vi "SMR_LabVIEW_V10.vi"() -> ()   [LabVIEW 2025]
uses:
  <vilib>/DAQmx/write.llb/DAQmx Write (Analog DBL 1Chan 1Samp).vi
  <vilib>/DAQmx/read.llb/DAQmx Read (Analog 1D DBL NChan 1Samp).vi
  <vilib>/DAQmx/read.llb/DAQmx Read (Analog 2D DBL NChan NSamp).vi
  <vilib>/Analysis/baseanly.llb/Mean (DBL).vi
  <vilib>/DAQmx/create/channels.llb/DAQmx Create Channel (AI-Temperature-Thermocouple).vi
  <vilib>/DAQmx/create/channels.llb/DAQmx Create Channel (AI-Voltage-Basic).vi
  <vilib>/DAQmx/create/channels.llb/DAQmx Create Channel (AO-Voltage-Basic).vi
  <vilib>/DAQmx/miscellaneous.llb/DAQmx Fill In Error Info.vi
  <vilib>/DAQmx/configure/timing.llb/DAQmx Timing (Sample Clock).vi
  <vilib>/DAQmx/create/channels.llb/DAQmx Create Channel (AO-Current-Basic).vi
  <vilib>/addons/control/pid/pid.llb/PID (DBL).vi
  <vilib>/measure/maspectr.llb/FFT Power Spectrum and PSD for 1 Chan.vi
  <vilib>/measure/matone.llb/Extract Single Tone Information 1 Chan.vi
  <vilib>/addons/control/pid/pid.llb/PID Advanced (DBL).vi
  <vilib>/addons/control/pid/NI_PID_pid.lvlib
  <vilib>/Analysis/NI_AALBase.lvlib
  <vilib>/ptbypt/NI_PtbyPt.lvlib
  <vilib>/measure/NI_MAPro.lvlib
panel:
  out "HX Flow (GPM)":dbl
  out "HW Valve Command (V)":dbl
  in  "HX Flow Setpoint (GPM)":dbl
  in  "Manual HW Valve Command (V)":dbl min=0.0 max=10.0
  in  "HW Valve: Manual / PID (on)":bool
  out "Rod Power (W)":dbl
  in  "Resistance Burden (Ohm)":dbl=220.0 min=220.0 max=220.0
  out "PSU Command (mA)":dbl
  in  "PSU Power Setpoint (W)":dbl
  in  "Manual PSU Command (0-8.8)":dbl min=0.0 max=8.8
  in  "PSU: Manual/ PID (on)":bool
  in  "PID gains for PSU":T1={"proportional gain (Kc)"=0.0003, "integral time (Ti, min)"=0.025, "derivative time (Td, min)"=0.0} {"derivative time (Td, min)" format="%.3f"; "integral time (Ti, min)" format="%.3f"; "proportional gain (Kc)" format="%.5f"}
  out "Room Temp (deg C)":dbl
  in  "PID gains for HW Valve":T1={"proportional gain (Kc)"=1.5, "integral time (Ti, min)"=0.35, "derivative time (Td, min)"=0.0} {"derivative time (Td, min)" format="%.3f"; "integral time (Ti, min)" format="%.3f"; "proportional gain (Kc)" format="%.3f"}
  out "Rod Power (W)":dbl
  out "Current Through Rod (A)":dbl
  out "Time in Steady State (s)":dbl
  in  "Steady-State Dwell (s)":dbl
  out "Main Loop Flow (GPM)":dbl
  out "FM Amplitude":dbl
  out "FM Frequency":dbl
  out "Spectrum":cluster{"f0":dbl, "df":dbl, "magnitude":dbl[]}(graph)
  out "Raw Signal":waveform(dbl)(graph)
  out "Smoothed HX Flow (GPM)":dbl
  out "Flow History":dbl(graph)
  out "HX Flow (GPM)":dbl
  out "Voltage Across Rod (V)":dbl format="%0.2f"
  out "Current Run Folder":path
  in  "Log Root Folder":path=path "C:/Users/LocalUser/Documents/GitHub/thermal-loop/resources/v0.1.1/data/001"
  out "Raw NI9201 \nVoltage Display":T2
  in  "Loop Period (ms)":dbl=1000.0
  in  "Stop":bool
  out "Auto Steady State Threshold (deg C/min)":dbl
  out "Max dT/dt (deg C/min)":dbl
  out "Temp Change Rate (deg C/min)":dbl
  out "5-Min Baseline Complete":bool
  out "Rate Window Ready":bool
  out "Steady State":bool
  in  "Voltage Limit (V)":dbl=10.0
  in  "Temperature Limit (C)":dbl=50.0
  in  "Pressure Limit (psi)":dbl=15.0
  out "Max Voltage":bool
  out "Max Temperature":bool
  out "Max Pressure":bool
  out "Heat Exchanger Pressure History":dbl(graph)
  out "Main Loop Pressure History":T3(graph)
  out "Overall Avg Pressure (psi)":dbl
  out "Heat Exchanger Pressure P6 (psi)":dbl
  out "Main Loop Avg Pressure (psi)":dbl
  out "Pressure Display":T4
  out "Overall Pressure History":T5(graph)
  out "Max Loop Pressure (psi)":dbl
  out "Heat Exchanger Temperature History":cluster{"Waveform":dbl, "Waveform":dbl}(graph)
  out "Main Loop Temeperature History":T6(graph)
  out "Heat Exchanger Avg Temp (deg C)":dbl
  out "Temperature Display":T7
  out "Overall Temperature History":T8(graph)
  out "Overall Avg Temp (deg C)":dbl
  out "Max Loop Temp (deg C)":dbl
  out "Final P-Valve Voltage (V)":dbl
  out "PID Trim Voltage (V)":dbl
  in  "PID Temp Setpoint (deg C)":dbl
  in  "Auto PID Enable":bool
  in  "Manual P-Valve Voltage (V)":dbl min=0.0 max=10.0
  out "Main Loop Avg Temp (deg C)":dbl
  # "HoneyWell Valve Control"
  # "PSU Control"
  # "Heat Exchanger Flow"
  # "Control/Troubleshoot"
  # "Steady State"
  # "Emergency Indicators"
  # "Pressure"
  # "Temperature"
  # "Proportional Valve Control"
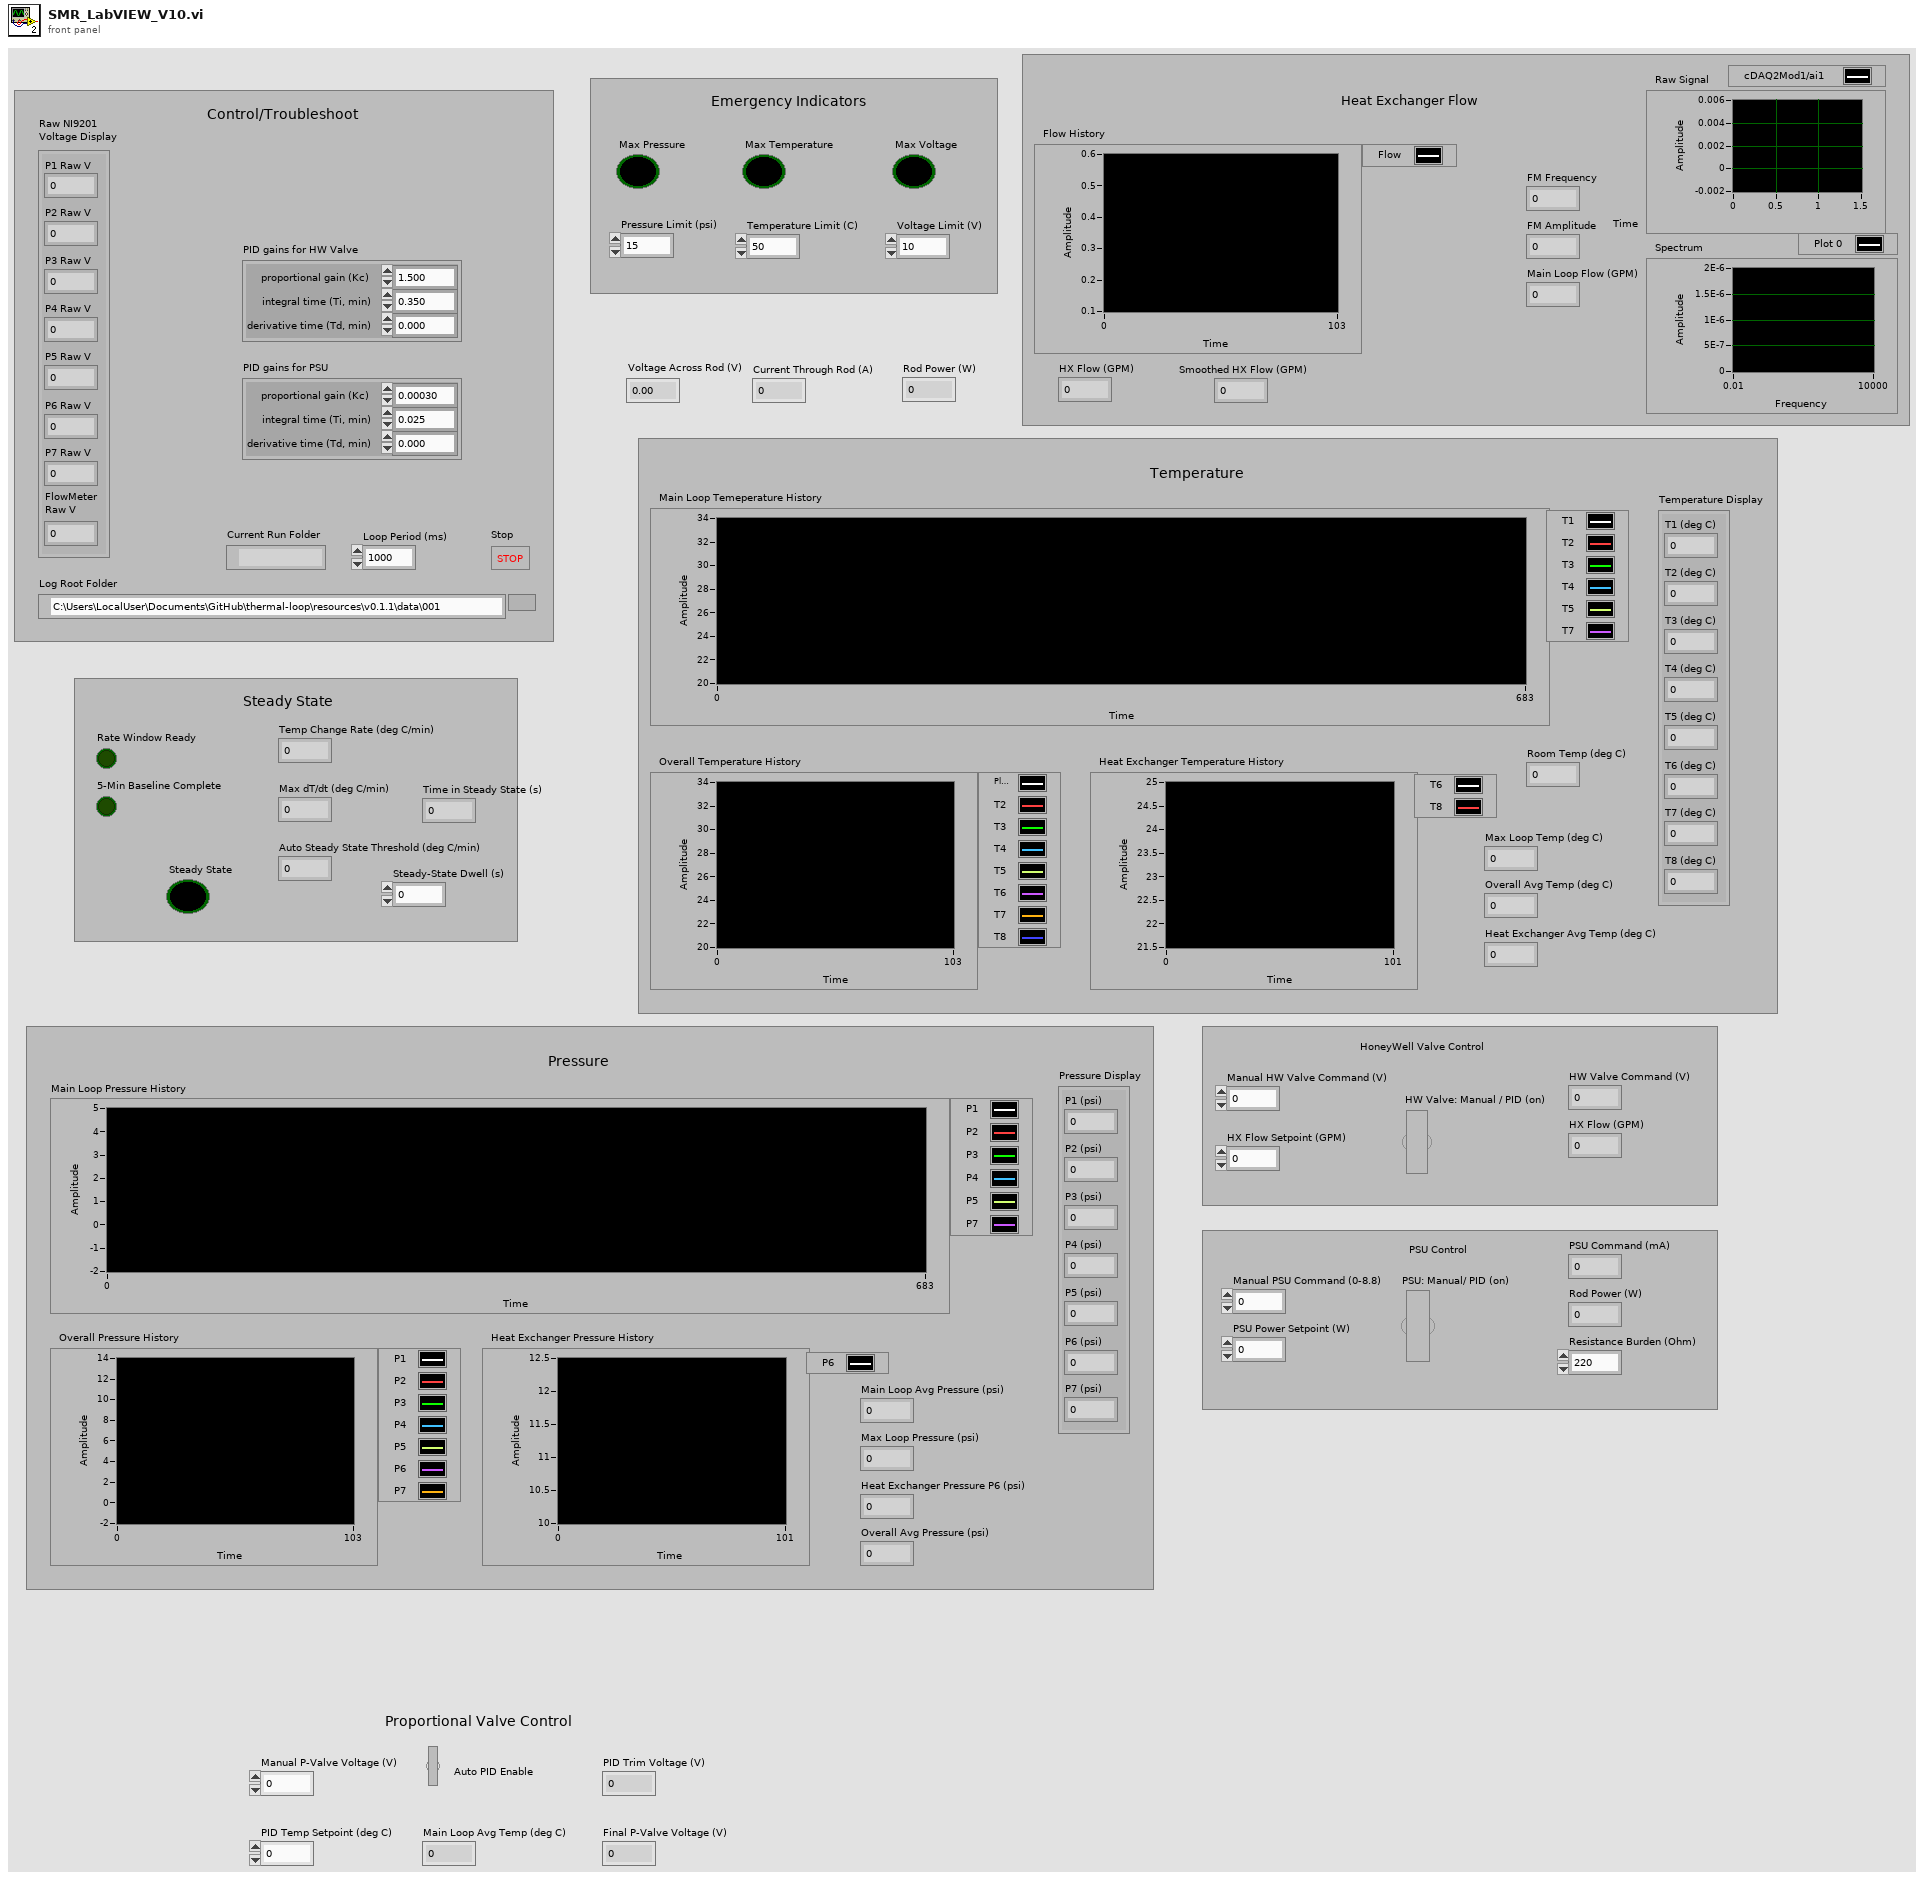
[diagram p1: front panel]
types:
  T1 = cluster{"proportional gain (Kc)":dbl, "integral time (Ti, min)":dbl, "derivative time (Td, min)":dbl}
  T2 = cluster{"P1 Raw V":dbl, "P2 Raw V":dbl, "P3 Raw V":dbl, "P4 Raw V":dbl, "P5 Raw V":dbl, "P6 Raw V":dbl, "P7 Raw V":dbl, "FlowMeter\nRaw V":dbl}
  T3 = cluster{"P1":dbl, "P2":dbl, "P3":dbl, "P4":dbl, "P5":dbl, "P7":dbl}
  T4 = cluster{"P1 (psi)":dbl, "P2 (psi)":dbl, "P3 (psi)":dbl, "P4 (psi)":dbl, "P5 (psi)":dbl, "P6 (psi)":dbl, "P7 (psi)":dbl}
  T5 = cluster{"P1":dbl, "P2":dbl, "P3":dbl, "P4":dbl, "P5":dbl, "P6":dbl, "P7":dbl}
  T6 = cluster{"Waveform":dbl, "Waveform":dbl, "Waveform":dbl, "Waveform":dbl, "Waveform":dbl, "Waveform":dbl}
  T7 = cluster{"T1 (deg C)":dbl, "T2 (deg C)":dbl, "T3 (deg C)":dbl, "T4 (deg C)":dbl, "T5 (deg C)":dbl, "T6 (deg C)":dbl, "T7 (deg C)":dbl, "T8 (deg C)":dbl}
  T8 = cluster{"Waveform":dbl, "Waveform":dbl, "Waveform":dbl, "Waveform":dbl, "Waveform":dbl, "Waveform":dbl, "Waveform":dbl, "Waveform":dbl}
  T9 = enum16{"open", "replace", "create", "open or create", "replace or create", "replace or create with confirmation"}
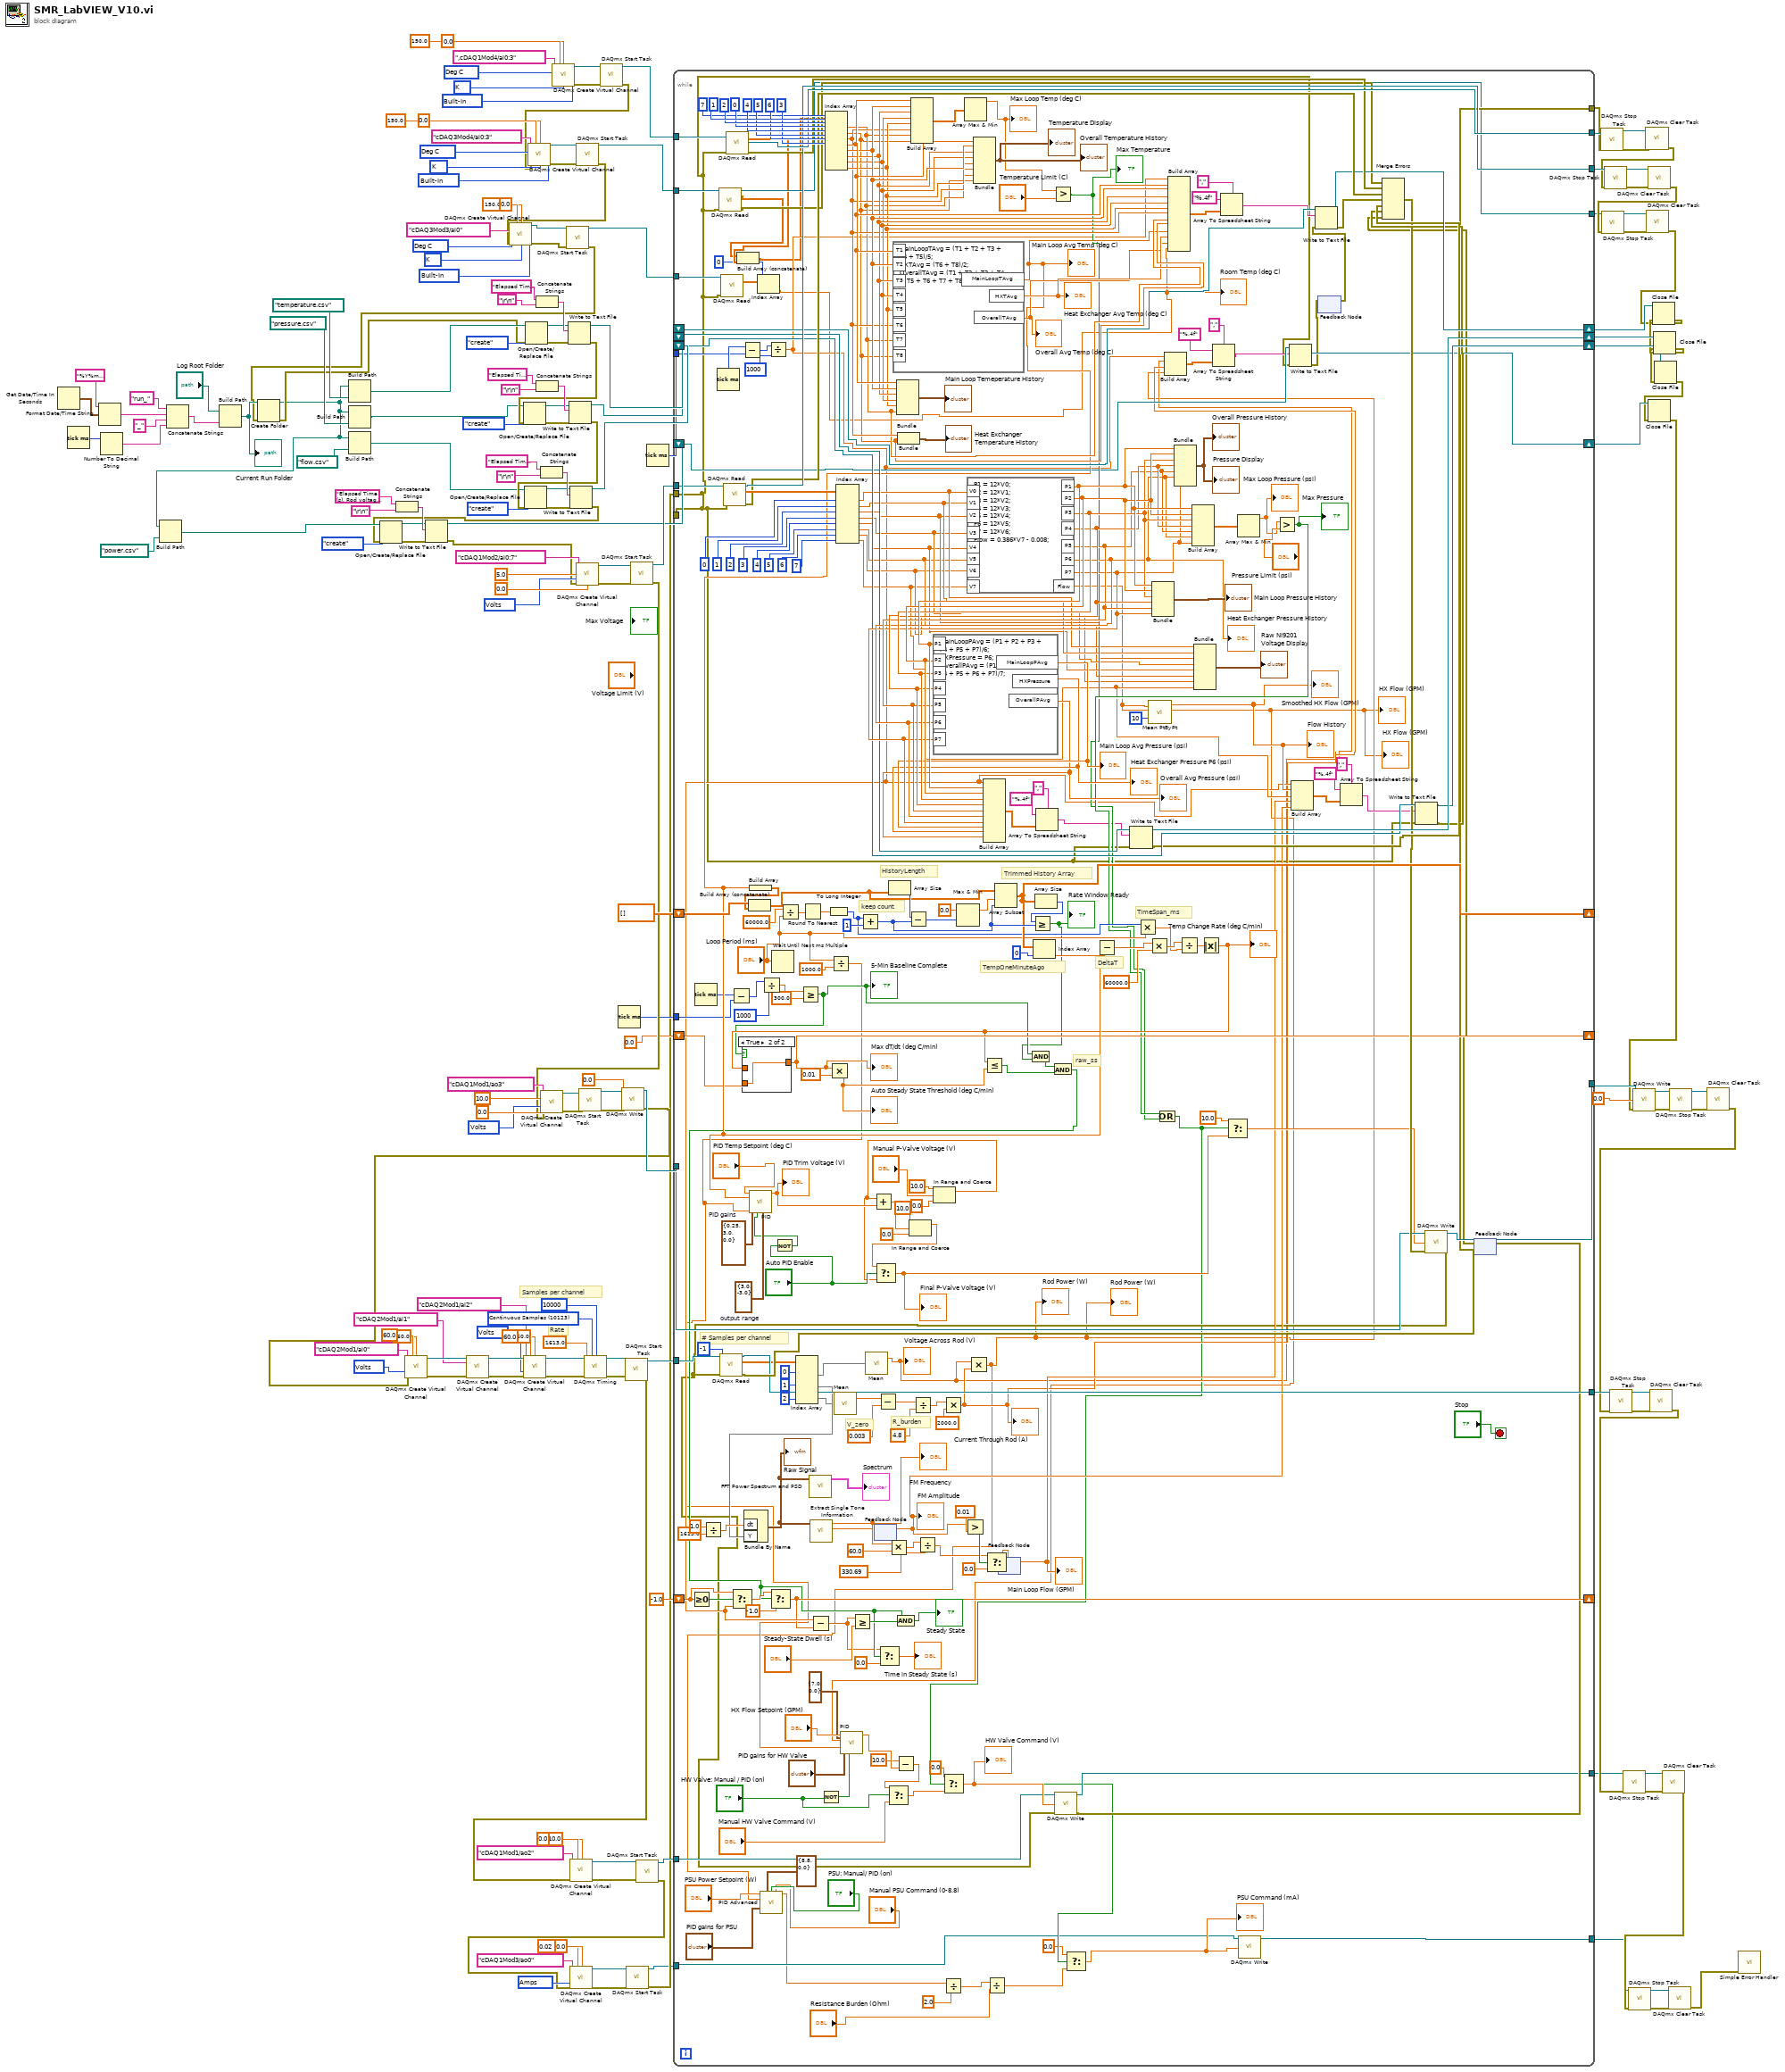
[diagram p0: block diagram]
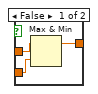
[diagram p2: hidden frame]
diagram:
  w9 = 10342 items=["Amps"=10342, "From Custom Scale"=10065] ("units")
  w15 = 10200 items=["Built-In"=10200, "Constant Value"=10116, "Channel"=10113] ("cjc source")
  w16 = 10073 items=["J"=10072, "K"=10073, "N"=10077, "R"=10082, "S"=10085, "T"=10086, "B"=10047, "E"=10055] ("thermocouple type")
  w22 = 10143 items=["Deg C"=10143, "Deg F"=10144, "Kelvins"=10325, "Deg R"=10145, "From Custom Scale"=10065] ("units")
  w40 = 10348 items=["Volts"=10348, "From Custom Scale"=10065] ("units")
  w56 = 10200 items=["Built-In"=10200, "Constant Value"=10116, "Channel"=10113] ("cjc source")
  w57 = 10073 items=["J"=10072, "K"=10073, "N"=10077, "R"=10082, "S"=10085, "T"=10086, "B"=10047, "E"=10055] ("thermocouple type")
  w58 = 10143 items=["Deg C"=10143, "Deg F"=10144, "Kelvins"=10325, "Deg R"=10145, "From Custom Scale"=10065] ("units")
  w88 = 10123 items=["Finite Samples"=10178, "Continuous Samples"=10123, "Hardware Timed Single Point"=12522] ("sample mode")
  w90 = 10348 items=["Volts"=10348, "From Custom Scale"=10065] ("units")
  w109 = 10348 items=["Volts"=10348, "From Custom Scale"=10065] ("units")
  w171 = 10200 items=["Built-In"=10200, "Constant Value"=10116, "Channel"=10113] ("cjc source")
  w172 = 10073 items=["J"=10072, "K"=10073, "N"=10077, "R"=10082, "S"=10085, "T"=10086, "B"=10047, "E"=10055] ("thermocouple type")
  w173 = 10143 items=["Deg C"=10143, "Deg F"=10144, "Kelvins"=10325, "Deg R"=10145, "From Custom Scale"=10065] ("units")
  w180 = 10348 items=["Volts"=10348, "From Custom Scale"=10065] ("units")
  # "Samples per channel"
  # "Rate"
  n1 = Get Date/Time In Seconds() -> (seconds since 1Jan1904=w130:timestamp)
  n2 = Tick Count (ms)() -> (millisecond timer value=w128:u32)
  n3 = Format Date/Time String(time format string (%c)="%Y%m%d_%H%M%S", seconds (now)=w130) -> (date/time string=w125:string)  [unwired: 1 in]
  n4 = Number To Decimal String(number=w128) -> (decimal integer string=w126:string)  [unwired: 1 in]
  n5 = Concatenate Strings("run_" ("string"), w125, "_" ("string"), w126) -> (w122:string)
  n6 = Build Path(base path="Log Root Folder", name or relative path=w122) -> (appended path=w121:path)
  "Current Run Folder" <- w121
  n7 = Concatenate Strings("Elapsed Time (s), Rod voltage (V), Rod Current (A), Rod Power (W)", "\r\n") -> (w75:string)
  n8 = Concatenate Strings("Elapsed Time (s),T1 (deg C),T2 (deg C),T3 (deg C),T4 (deg C),T5 (deg C),T6 (deg C),T7 (deg C),T8 (deg C),Main Loop Avg Temp (deg C),HX Avg Temp (deg C),Overall Avg Temp (deg C), Room Temp (deg C)", "\r\n") -> (w154:string)
  n9 = Concatenate Strings("Elapsed Time (s),P1 (psi),P2 (psi),P3 (psi),P4 (psi),P5 (psi),P6 (psi),P7 (psi),Main Loop Avg Pressure (psi),HX Pressure (psi),Overall Avg Pressure (psi)", "\r\n") -> (w152:string)
  n10 = Concatenate Strings("Elapsed Time (s),Heat Exchanger Flow (GPM),Flow Raw Voltage (V), Main Loop Flow (GPM), Flow Signal Amplitude (V)", "\r\n") -> (w148:string)
  n11 = call-poly <vilib>:"DAQmx Create Virtual Channel.vi"("maximum value"=150.0, "minimum value"=0.0, "physical channels"=tag ",cDAQ1Mod4/ai0:3", "cjc source"=w171, "units"=w173, "thermocouple type"=w172) -> ("task out"=w170:refnum<k21>, "error out"=w169:errorcluster)  [unwired: 8 in]
  n12 = call <vilib>:"DAQmx Start Task.vi"("task/channels in"=w170, "error in"=w169) -> ("task out"=w168:refnum<k21>, "error out"=w52:errorcluster)  [unwired: 12 in]
  n13 = call-poly <vilib>:"DAQmx Create Virtual Channel.vi"("maximum value"=150.0, "minimum value"=0.0, "physical channels"=tag "cDAQ3Mod4/ai0:3", "cjc source"=w56, "units"=w58, "error in"=w52, "thermocouple type"=w57) -> ("task out"=w55:refnum<k21>, "error out"=w54:errorcluster)  [unwired: 7 in]
  n14 = call <vilib>:"DAQmx Start Task.vi"("task/channels in"=w55, "error in"=w54) -> ("task out"=w51:refnum<k21>, "error out"=w19:errorcluster)  [unwired: 12 in]
  n15 = call-poly <vilib>:"DAQmx Create Virtual Channel.vi"("maximum value"=150.0, "minimum value"=0.0, "physical channels"=tag "cDAQ3Mod3/ai0", "cjc source"=w15, "units"=w22, "error in"=w19, "thermocouple type"=w16) -> ("task out"=w21:refnum<k21>, "error out"=w20:errorcluster)  [unwired: 7 in]
  n16 = call <vilib>:"DAQmx Start Task.vi"("task/channels in"=w21, "error in"=w20) -> ("task out"=w17:refnum<k21>, "error out"=w18:errorcluster)  [unwired: 12 in]
  n17 = Create Folder(path (use dialog)=w121, error in=w18) -> (created path=w69:path, error out=w114:errorcluster)  [unwired: 1 in, 1 out]
  n18 = Build Path(base path=w69, name or relative path=path "power.csv") -> (appended path=w70:path)
  n19 = Build Path(base path=w69, name or relative path=path "temperature.csv") -> (appended path=w120:path)
  n20 = Build Path(base path=w69, name or relative path=path "pressure.csv") -> (appended path=w119:path)
  n21 = Build Path(base path=w69, name or relative path=path "flow.csv") -> (appended path=w118:path)
  n22 = Open/Create/Replace File(file path (use dialog)=w120, error in=w114, operation (0:open)=T9."create") -> (refnum out=w153:refnum<file>, error out=w137:errorcluster)  [unwired: 3 in, 1 out]
  n23 = Write to Text File(file (use dialog)=w153, text=w154, error in=w137) -> (refnum out=w144:refnum<file>, error out=w136:errorcluster)  [unwired: 1 in, 1 out]
  n24 = Open/Create/Replace File(file path (use dialog)=w119, error in=w136, operation (0:open)=T9."create") -> (refnum out=w151:refnum<file>, error out=w135:errorcluster)  [unwired: 3 in, 1 out]
  n25 = Write to Text File(file (use dialog)=w151, text=w152, error in=w135) -> (refnum out=w143:refnum<file>, error out=w134:errorcluster)  [unwired: 1 in, 1 out]
  n26 = Open/Create/Replace File(file path (use dialog)=w118, error in=w134, operation (0:open)=T9."create") -> (refnum out=w147:refnum<file>, error out=w133:errorcluster)  [unwired: 3 in, 1 out]
  n27 = Write to Text File(file (use dialog)=w147, text=w148, error in=w133) -> (refnum out=w142:refnum<file>, error out=w67:errorcluster)  [unwired: 1 in, 1 out]
  n28 = Open/Create/Replace File(file path (use dialog)=w70, error in=w67, operation (0:open)=T9."create") -> (refnum out=w74:refnum<file>, error out=w71:errorcluster)  [unwired: 3 in, 1 out]
  n29 = Write to Text File(file (use dialog)=w74, text=w75, error in=w71) -> (refnum out=w65:refnum<file>, error out=w66:errorcluster)  [unwired: 1 in, 1 out]
  n30 = call-poly <vilib>:"DAQmx Create Virtual Channel.vi"("maximum value"=5.0, "minimum value"=0.0, "physical channels"=tag "cDAQ1Mod2/ai0:7", "units"=w180, "error in"=w66) -> ("task out"=w179:refnum<k21>, "error out"=w178:errorcluster)  [unwired: 9 in]
  n31 = Tick Count (ms)() -> (millisecond timer value=w95:u32)
  n32 = call <vilib>:"DAQmx Start Task.vi"("task/channels in"=w179, "error in"=w178) -> ("task out"=w177:refnum<k21>, "error out"=w102:errorcluster)  [unwired: 12 in]
  n33 = call-poly <vilib>:"DAQmx Create Virtual Channel.vi"("maximum value"=10.0, "minimum value"=0.0, "physical channels"=tag "cDAQ1Mod1/ao3", "units"=w109, "error in"=w102) -> ("task out"=w108:refnum<k21>, "error out"=w107:errorcluster)  [unwired: 9 in]
  n34 = call <vilib>:"DAQmx Start Task.vi"("task/channels in"=w108, "error in"=w107) -> ("task out"=w106:refnum<k21>, "error out"=w105:errorcluster)  [unwired: 12 in]
  n35 = call-poly <vilib>:"DAQmx Write.vi"("task/channels in"=w106, "data"=0.0, "error in"=w105) -> ("task out"=w103:refnum<k21>, "error out"=w82:errorcluster)  [unwired: 10 in, 1 out]
  n36 = call-poly <vilib>:"DAQmx Create Virtual Channel.vi"("maximum value"=60.0, "minimum value"=-60.0, "physical channels"=tag "cDAQ2Mod1/ai0", "units"=w90, "error in"=w82) -> ("task out"=w79:refnum<k21>, "error out"=w78:errorcluster)  [unwired: 9 in]
  n37 = call-poly <vilib>:"DAQmx Create Virtual Channel.vi"("task in"=w79, "physical channels"=tag "cDAQ2Mod1/ai1", "error in"=w78) -> ("task out"=w44:refnum<k21>, "error out"=w42:errorcluster)  [unwired: 11 in]
  n38 = call-poly <vilib>:"DAQmx Create Virtual Channel.vi"("task in"=w44, "maximum value"=60.0, "minimum value"=-60.0, "physical channels"=tag "cDAQ2Mod1/ai2", "units"=w40, "error in"=w42) -> ("task out"=w43:refnum<k21>, "error out"=w41:errorcluster)  [unwired: 8 in]
  n39 = call-poly <vilib>:"DAQmx Timing.vi"("task/channels in"=w43, "sample mode"=w88, "samples per channel"=10000, "rate"=1613.0, "error in"=w41) -> ("task out"=w86:refnum<k21>, "error out"=w85:errorcluster)  [unwired: 9 in]
  n40 = call <vilib>:"DAQmx Start Task.vi"("task/channels in"=w86, "error in"=w85) -> ("task out"=w81:refnum<k21>, "error out"=w31:errorcluster)  [unwired: 12 in]
  n41 = call-poly <vilib>:"DAQmx Create Virtual Channel.vi"("maximum value"=10.0, "minimum value"=0.0, "physical channels"=tag "cDAQ1Mod1/ao2", "error in"=w31) -> ("task out"=w34:refnum<k21>, "error out"=w33:errorcluster)  [unwired: 10 in]
  n42 = call <vilib>:"DAQmx Start Task.vi"("task/channels in"=w34, "error in"=w33) -> ("task out"=w32:refnum<k21>, "error out"=w8:errorcluster)  [unwired: 12 in]
  n43 = call-poly <vilib>:"DAQmx Create Virtual Channel.vi"("maximum value"=0.02, "minimum value"=0.0, "physical channels"=tag "cDAQ1Mod3/ao0", "units"=w9, "error in"=w8) -> ("task out"=w14:refnum<k21>, "error out"=w13:errorcluster)  [unwired: 9 in]
  n44 = call <vilib>:"DAQmx Start Task.vi"("task/channels in"=w14, "error in"=w13) -> ("task out"=w1:refnum<k21>, "error out"=w7:errorcluster)  [unwired: 12 in]
  n45 = Tick Count (ms)() -> (millisecond timer value=w141:u32)
  n46 = while {
    tunnel: w177 -> [w437]
    tunnel: w168 -> [w420]
    tunnel: [w411] -> w167
    tunnel: [w204] -> _
    tunnel: [w410] -> w166
    tunnel: [w298] -> w165
    shift-right: [w389] -> w140
    shift-left: w144 -> [w390]
    shift-right: [w374] -> w139
    shift-left: w143 -> [w375]
    shift-right: [w369] -> w138
    shift-left: w142 -> [w370]
    tunnel: w141 -> [w406]
    shift-right: [w348] -> _
    shift-left: dbl[] [] -> [w361]
    tunnel: w103 -> [w330]
    tunnel: w7 -> [w204]
    tunnel: [w336] -> w100
    tunnel: w95 -> [w319]
    shift-right: [w312] -> _
    shift-left: 0.0 -> [w314]
    tunnel: w81 -> [w297]
    tunnel: [w296] -> w80
    shift-right: [w259] -> w64
    shift-left: w65 -> [w260]
    shift-right: [w251] -> _
    shift-left: -1.0 -> [w255]
    tunnel: w51 -> [w243]
    tunnel: [w241] -> w47
    tunnel: w32 -> [w223]
    tunnel: [w219] -> w26
    tunnel: w17 -> [w205]
    tunnel: [w194] -> w2
    tunnel: w1 -> [w193]
    stop <- "Stop" stop-if-true
    w334 = cluster{"output high":dbl, "output low":dbl} {"output high"=3.0, "output low"=-3.0}  # output range
    w335 = T1 {"proportional gain (Kc)"=0.25, "integral time (Ti, min)"=3.0, "derivative time (Td, min)"=0.0}  # PID gains
    # "R_burden"
    # "V_zero"
    # "raw_ss"
    # "# Samples per channel"
    # "TimeSpan_ms"
    # "DeltaT"
    # "TempOneMinuteAgo"
    # "Trimmed History Array"
    # "HistoryLength"
    # "keep count"
    n47 = Greater Or Equal To 0?(x=w255) -> (x >= 0?=w256:bool)
    n48 = Tick Count (ms)() -> (millisecond timer value=w320:u32)
    n49 = Divide(x=1.0, y=1613.0) -> (x/y=w270:dbl)
    n50 = Tick Count (ms)() -> (millisecond timer value=w407:u32)
    n51 = call-poly <vilib>:"DAQmx Read.vi"("task/channels in"=w243, "error in"=w204) -> ("task out"=w241:refnum<k21>, "data"=w238:dbl[], "error out"=w242:errorcluster)  [unwired: 11 in]
    n52 = call-poly <vilib>:"DAQmx Read.vi"("task/channels in"=w205, "error in"=w204) -> ("data"=w202:dbl[])  [unwired: 11 in, 2 out]
    n53 = call-poly <vilib>:"DAQmx Read.vi"("task/channels in"=w437, "error in"=w204) -> ("task out"=w410:refnum<k21>, "data"=w428:dbl[], "error out"=w408:errorcluster)  [unwired: 11 in]
    n54 = call-poly <vilib>:"DAQmx Read.vi"("task/channels in"=w420, "error in"=w204) -> ("task out"=w411:refnum<k21>, "data"=w239:dbl[], "error out"=w409:errorcluster)  [unwired: 11 in]
    n55 = Subtract(x=w320, y=w319) -> (x-y=w318:u32)
    n56 = Build Array (concatenate)(w238, w239) -> (w240:dbl[])
    n57 = Subtract(x=w407, y=w406) -> (x-y=w405:u32)
    n58 = Index Array(array=w202, index=0) -> (element=w201:dbl)
    "Room Temp (deg C)" <- w201
    n59 = Divide(x=w318, y=u32 1000) -> (x/y=w316:dbl)
    n60 = Divide(x=w405, y=u32 1000) -> (x/y=w252:dbl)
    n61 = Select(t=w255, s=w256, f=w252) -> (s? t:f=w254:dbl)
    n62 = Wait Until Next ms Multiple(millisecond multiple="Loop Period (ms)") -> ()  [unwired: 1 out]
    n63 = Not(x="Auto PID Enable") -> (.not. x?=w331:bool)
    n64 = Divide(x=60000.0, y="Loop Period (ms)") -> (x/y=w358:dbl)
    n65 = Greater Or Equal?(x=w316, y=300.0) -> (x >= y?=w309:bool)
    "5-Min Baseline Complete" <- w309
    n66 = Round To Nearest(number=w358) -> (nearest integer value=w357:dbl)
    n67 = Not(x="HW Valve: Manual / PID (on)") -> (.not. x?=w232:bool)
    n68 = Index Array(array=w240, index #1=7 ("index"), index #2=1 ("index"), index #3=2 ("index"), index #4=0 ("index"), index #5=4 ("index"), index #6=5 ("index"), index #7=6 ("index"), index #8=3 ("index")) -> (element #1=w397:dbl, element #2=w396:dbl, element #3=w398:dbl, element #4=w403:dbl, element #5=w402:dbl, element #6=w401:dbl, element #7=w400:dbl, element #8=w399:dbl)
    n69 = To Long Integer(number=w357) -> (32bit integer=w345:i32)
    n70 = Divide(x="Loop Period (ms)", y=1000.0) -> (x/y=w218:dbl)
    n71 = Index Array(array=w428, index #1=0 ("index"), index #2=1 ("index"), index #3=2 ("index"), index #4=3 ("index"), index #5=4 ("index"), index #6=5 ("index"), index #7=6 ("index"), index #8=7 ("index")) -> (element #1=w295:dbl, element #2=w294:dbl, element #3=w293:dbl, element #4=w292:dbl, element #5=w291:dbl, element #6=w290:dbl, element #7=w289:dbl, element #8=w288:dbl)
    n72 = Add(x=w345, y=1) -> (x+y=w350:i32)
    n73 = feedback #1() -> (w266:dbl)  [unwired: 1 in]
    "FM Amplitude" <- w266
    n74 = formula code="MainLoopTAvg = (T1 + T2 + T3 + T4 + T5)/5;\nHXTAvg = (T6 + T8)/2;\nOverallTAvg = (T1 + T2 + T3 + T4 + T5 + T6 + T7 + T8)/8;"("T1"=w403, "T2"=w402, "T3"=w401, "T4"=w400, "T5"=w399, "T6"=w398, "T7"=w397, "T8"=w396) -> ("MainLoopTAvg"=w322:dbl, "HXTAvg"=w395:dbl, "OverallTAvg"=w394:dbl)
    "Overall Avg Temp (deg C)" <- w394
    "Main Loop Avg Temp (deg C)" <- w322
    "Heat Exchanger Avg Temp (deg C)" <- w395
    n75 = Build Array(w322) -> (w360:dbl[])
    n76 = Build Array (concatenate)(w361, w360) -> (w352:dbl[])
    n77 = call-poly <vilib>:"PID.vi"("reinitialize? (F)"=w331, "output range"=w334, "dt (s)"=w218, "PID gains"=w335, "process variable"=w322, "setpoint"="PID Temp Setpoint (deg C)") -> ("output"=w329:dbl)  [unwired: 4 in, 1 out]
    "PID Trim Voltage (V)" <- w329
    n78 = Array Size(array=w352) -> (size(s)=w355:i32)
    n79 = Bundle("Waveform"=w403, "Waveform"=w402, "Waveform"=w401, "Waveform"=w400, "Waveform"=w399, "Waveform"=w397) -> (→"Main Loop Temeperature History":T6)  [unwired: 1 in]
    n80 = Bundle("Waveform"=w398, "Waveform"=w396) -> (→"Heat Exchanger Temperature History":cluster{"Waveform":dbl, "Waveform":dbl})  [unwired: 1 in]
    n81 = Subtract(x=w355, y=w350) -> (x-y=w353:i32)
    n82 = Build Array(w403, w402, w401, w400, w399, w398, w397, w396) -> (w438:dbl[])
    n83 = In Range and Coerce(upper limit=10.0, x="Manual P-Valve Voltage (V)", lower limit=0.0) -> (coerced(x)=w324:dbl)  [unwired: 1 out]
    n84 = Add(x=w324, y=w329) -> (x+y=w328:dbl)
    n85 = In Range and Coerce(upper limit=10.0, x=w328, lower limit=0.0) -> (coerced(x)=w323:dbl)  [unwired: 1 out]
    n86 = Select(t=w323, s="Auto PID Enable", f=w324) -> (s? t:f=w301:dbl)
    "Final P-Valve Voltage (V)" <- w301
    n87 = Max & Min(x=0.0, y=w353) -> (max(x,y)=w351:dbl)  [unwired: 1 out]
    n88 = Array Max & Min(array=w438) -> (max value=w363:dbl)  [unwired: 3 out]
    "Max Loop Temp (deg C)" <- w363
    n89 = Greater?(x=w266, y=0.01) -> (0:w274:bool)
    n90 = formula code="P1 = 12*V0;\nP2 = 12*V1;\nP3 = 12*V2;\nP4 = 12*V3;\nP5 = 12*V4;\nP6 = 12*V5; \nP7 = 12*V6;\nFlow = 0.386*V7 - 0.008;"("V0"=w295, "V1"=w294, "V2"=w293, "V3"=w292, "V4"=w291, "V5"=w290, "V6"=w289, "V7"=w288) -> ("P1"=w388:dbl, "P2"=w387:dbl, "P3"=w386:dbl, "P4"=w385:dbl, "P5"=w384:dbl, "P6"=w383:dbl, "P7"=w382:dbl, "Flow"=w184:dbl)
    "HX Flow (GPM)" <- w184
    "Heat Exchanger Pressure History" <- w383
    "HX Flow (GPM)" <- w184
    n91 = call-poly <vilib>:"PID.vi"("reinitialize? (F)"=w232, "output range"=cluster{"output high":dbl, "output low":dbl} {"output high"=7.0, "output low"=0.0}, "dt (s)"=w218, "PID gains"="PID gains for HW Valve", "process variable"=w184, "setpoint"="HX Flow Setpoint (GPM)") -> ("output"=w231:dbl)  [unwired: 4 in, 1 out]
    n92 = Subtract(x=10.0, y=w231) -> (x-y=w228:dbl)
    n93 = Select(t=w228, s="HW Valve: Manual / PID (on)", f="Manual HW Valve Command (V)") -> (s? t:f=w226:dbl)
    n94 = formula code="MainLoopPAvg = (P1 + P2 + P3 + P4 + P5 + P7)/6;\nHXPressure = P6;\nOverallPAvg = (P1 + P2 + P3 + P4 + P5 + P6 + P7)/7;"("P1"=w388, "P2"=w387, "P3"=w386, "P4"=w385, "P5"=w384, "P6"=w383, "P7"=w382) -> ("MainLoopPAvg"=w381:dbl, "HXPressure"=w380:dbl, "OverallPAvg"=w379:dbl)
    "Overall Avg Pressure (psi)" <- w379
    "Heat Exchanger Pressure P6 (psi)" <- w380
    "Main Loop Avg Pressure (psi)" <- w381
    n95 = Bundle("Waveform"=w403, "Waveform"=w402, "Waveform"=w401, "Waveform"=w400, "Waveform"=w399, "Waveform"=w398, "Waveform"=w397, "Waveform"=w396) -> (→"Overall Temperature History" →"Temperature Display":T8)  [unwired: 1 in]
    n96 = Build Array(w252, w388, w387, w386, w385, w384, w383, w382, w381, w380, w379) -> (w378:dbl[])
    n97 = Array Subset(array=w352, index=w351, length=w350) -> (w348:dbl[])
    n98 = feedback #2() -> (w264:dbl)  [unwired: 1 in]
    "Main Loop Flow (GPM)" <- w264
    n99 = Index Array(array=w348, index=0) -> (element=w346:dbl)
    n100 = Array Size(array=w348) -> (size(s)=w349:i32)
    n101 = Greater Or Equal?(x=w349, y=w350) -> (x >= y?=w308:bool)
    "Rate Window Ready" <- w308
    n102 = And(x=w309, y=w308) -> (x .and. y?=w307:bool)
    n103 = Array To Spreadsheet String(delimiter (Tab)=",", array=w378, 3:"%.4f" ("format string")) -> (spreadsheet string=w214:string)
    n104 = Greater?(x=w363, y="Temperature Limit (C)") -> (0:w304:bool)
    "Max Temperature" <- w304
    n105 = Subtract(x=w322, y=w346) -> (x-y=w344:dbl)
    n106 = Write to Text File(file (use dialog)=w375, text=w214, error in=w204) -> (refnum out=w374:refnum<file>, error out=w367:errorcluster)  [unwired: 1 in, 1 out]
    n107 = Multiply(x=w345, y="Loop Period (ms)") -> (x*y=w341:dbl)
    n108 = Multiply(x=w344, y=60000.0) -> (x*y=w342:dbl)
    n109 = call <vilib>:"Mean PtByPt.vi"("x"=w184, "sample length"=10) -> ("mean"=w286:dbl)  [unwired: 2 in, 1 out]
    "Flow History" <- w286
    "Smoothed HX Flow (GPM)" <- w286
    n110 = Bundle("P1"=w388, "P2"=w387, "P3"=w386, "P4"=w385, "P5"=w384, "P7"=w382) -> (→"Main Loop Pressure History":T3)  [unwired: 1 in]
    n111 = Build Array(w252, w403, w402, w401, w400, w399, w398, w397, w396, w322, w395, w394, w201) -> (w393:dbl[])
    n112 = Bundle("P1"=w388, "P2"=w387, "P3"=w386, "P4"=w385, "P5"=w384, "P6"=w383, "P7"=w382) -> (→"Overall Pressure History" →"Pressure Display":T5)  [unwired: 1 in]
    n113 = Divide(x=w342, y=w341) -> (x/y=w340:dbl)
    n114 = Build Array(w388, w387, w386, w385, w384, w383, w382) -> (w427:dbl[])
    n115 = Bundle("Waveform"=w295, "Waveform"=w294, "Waveform"=w293, "Waveform"=w292, "Waveform"=w291, "Waveform"=w290, "Waveform"=w289, "Waveform"=w288) -> (→"Raw NI9201 \nVoltage Display":T8)  [unwired: 1 in]
    n116 = Absolute Value(x=w340) -> (abs(x)=w311:dbl)
    "Temp Change Rate (deg C/min)" <- w311
    n117 = case shown="True" w309 {
      tunnel: w314 -> [w442 w443]
      tunnel: w311 -> [w441 _]
      tunnel: [w440 w443] -> w312
      frame False {
        n118 = Max & Min(x=w441, y=w442) -> (max(x,y)=w440:dbl)  [unwired: 1 out]
      }
      frame True {
      }
    }
    "Max dT/dt (deg C/min)" <- w312
    n119 = Multiply(x=w312, y=0.01) -> (x*y=w310:dbl)
    "Auto Steady State Threshold (deg C/min)" <- w310
    n120 = Less Or Equal?(x=w311, y=w310) -> (x <= y?=w306:bool)
    n121 = And(x=w307, y=w306) -> (x .and. y?=w247:bool)
    n122 = Select(t=w254, s=w247, f=-1.0) -> (s? t:f=w251:dbl)
    n123 = Subtract(x=w252, y=w251) -> (x-y=w246:dbl)
    n124 = Greater Or Equal?(x=w246, y="Steady-State Dwell (s)") -> (x >= y?=w249:bool)
    n125 = Select(t=w246, s=w247, f=0.0) -> (s? t:f=→"Time in Steady State (s)":dbl)
    n126 = And(x=w247, y=w249) -> (x .and. y?=→"Steady State":bool)
    n127 = Array To Spreadsheet String(delimiter (Tab)=",", array=w393, 3:"%.4f" ("format string")) -> (spreadsheet string=w215:string)
    n128 = Array Max & Min(array=w427) -> (max value=w364:dbl)  [unwired: 3 out]
    "Max Loop Pressure (psi)" <- w364
    n129 = Greater?(x=w364, y="Pressure Limit (psi)") -> (0:w305:bool)
    "Max Pressure" <- w305
    n130 = Or(x=w305, y=w304) -> (x .or. y?=w197:bool)
    n131 = Select(t=0.0, s=w197, f=w226) -> (s? t:f=w224:dbl)
    "HW Valve Command (V)" <- w224
    n132 = Select(t=10.0, s=w197, f=w301) -> (s? t:f=w300:dbl)
    n133 = Build Array(w252, w286, w288, w264, w266) -> (w373:dbl[])
    n134 = feedback #3() -> (w257:errorcluster)  [unwired: 1 in]
    n135 = Write to Text File(file (use dialog)=w390, text=w215, error in=w257) -> (refnum out=w389:refnum<file>, error out=w368:errorcluster)  [unwired: 1 in, 1 out]
    n136 = Array To Spreadsheet String(delimiter (Tab)=",", array=w373, 3:"%.4f" ("format string")) -> (spreadsheet string=w217:string)
    n137 = Write to Text File(file (use dialog)=w370, text=w217, error in=w204) -> (refnum out=w369:refnum<file>, error out=w366:errorcluster)  [unwired: 1 in, 1 out]
    n138 = feedback #4() -> (w220:errorcluster)  [unwired: 1 in]
    n139 = Merge Errors(w242, w409, w408, w368, w367, w366, w220) -> (w337:errorcluster)
    n140 = call-poly <vilib>:"DAQmx Write.vi"("task/channels in"=w330, "data"=w300, "error in"=w337) -> ("task out"=w336:refnum<k21>, "error out"=w222:errorcluster)  [unwired: 10 in, 1 out]
    n141 = call-poly <vilib>:"DAQmx Read.vi"("task/channels in"=w297, "number of samples per channel"=-1, "error in"=w222) -> ("task out"=w296:refnum<k21>, "data"=w285:dbl[][], "error out"=w298:errorcluster)  [unwired: 10 in]
    n142 = Index Array(array=w285, index (row) #1=0 ("index (row)"), index (row) #2=1 ("index (row)"), index (row) #3=2 ("index (row)")) -> (element #1=w284:dbl[], element #2=w269:dbl[], element #3=w236:dbl[])  [unwired: 3 in]
    n143 = Bundle By Name("dt"=w270, "Y"=w269) -> (w268:waveform(dbl))  [unwired: 1 in]
    "Raw Signal" <- w268
    n144 = call-poly <vilib>:"FFT Power Spectrum and PSD.vi"("time signal"=w268) -> ("Power Spectrum / PSD"=→"Spectrum":cluster{"f0":dbl, "df":dbl, "magnitude":dbl[]})  [unwired: 7 in, 3 out]
    n145 = call-poly <vilib>:"Extract Single Tone Information.vi"("time signal in"=w268) -> ("detected amplitude"=w267:dbl, "detected frequency"=w280:dbl)  [unwired: 5 in, 4 out]
    "FM Frequency" <- w280
    n146 = call-poly <vilib>:"Mean.vi"("X"=w236) -> ("mean"=w213:dbl)  [unwired: 1 out]
    n147 = call-poly <vilib>:"Mean.vi"("X"=w284) -> ("mean"=w206:dbl)  [unwired: 1 out]
    "Voltage Across Rod (V)" <- w206
    n148 = feedback-in #1(w267) -> ()
    n149 = Subtract(x=w213, y=0.003) -> (x-y=w211:dbl)
    n150 = Multiply(x=w280, y=60.0) -> (x*y=w278:dbl)
    n151 = Divide(x=w211, y=4.8) -> (x/y=w209:dbl)
    n152 = Divide(x=w278, y=330.69) -> (x/y=w273:dbl)
    n153 = Multiply(x=w209, y=2000.0) -> (x*y=w207:dbl)
    "Current Through Rod (A)" <- w207
    n154 = Multiply(x=w206, y=w207) -> (x*y=w185:dbl)
    "Rod Power (W)" <- w185
    "Rod Power (W)" <- w185
    n155 = call-poly <vilib>:"PID Advanced.vi"("setpoint"="PSU Power Setpoint (W)", "output range"=cluster{"output high":dbl, "output low":dbl} {"output high"=8.8, "output low"=0.0}, "auto? (T)"="PSU: Manual/ PID (on)", "manual control"="Manual PSU Command (0-8.8)", "process variable"=w185, "PID gains"="PID gains for PSU") -> ("output"=w187:dbl)  [unwired: 8 in, 1 out]
    n156 = Divide(x=w187, y=2.0) -> (x/y=w198:dbl)
    n157 = Select(t=w273, s=w274, f=0.0) -> (s? t:f=w265:dbl)
    n158 = Divide(x=w198, y="Resistance Burden (Ohm)") -> (x/y=w196:dbl)
    n159 = feedback-in #2(w265) -> ()
    n160 = call-poly <vilib>:"DAQmx Write.vi"("task/channels in"=w223, "data"=w224, "error in"=w222) -> ("task out"=w219:refnum<k21>, "error out"=w221:errorcluster)  [unwired: 10 in, 1 out]
    n161 = Select(t=0.0, s=w197, f=w196) -> (s? t:f=w200:dbl)
    "PSU Command (mA)" <- w200
    n162 = Build Array(w252, w206, w207, w185) -> (w261:dbl[])
    n163 = Array To Spreadsheet String(delimiter (Tab)=",", array=w261, 3:"%.4f" ("format string")) -> (spreadsheet string=w216:string)
    n164 = call-poly <vilib>:"DAQmx Write.vi"("task/channels in"=w193, "data"=w200) -> ("task out"=w194:refnum<k21>)  [unwired: 11 in, 2 out]
    n165 = Write to Text File(file (use dialog)=w260, text=w216, error in=w204) -> (refnum out=w259:refnum<file>, error out=w258:errorcluster)  [unwired: 1 in, 1 out]
    n166 = feedback-in #3(w258) -> ()
    n167 = feedback-in #4(w221) -> ()
  }
  n168 = call <vilib>:"DAQmx Stop Task.vi"("task/channels in"=w167, "error in"=w165) -> ("task out"=w164:refnum<k21>, "error out"=w162:errorcluster)  [unwired: 12 in]
  n169 = call <vilib>:"DAQmx Clear Task.vi"("task in"=w164, "error in"=w162) -> ("error out"=w161:errorcluster)  [unwired: 13 in]
  n170 = call <vilib>:"DAQmx Stop Task.vi"("task/channels in"=w166, "error in"=w161) -> ("task out"=w163:refnum<k21>, "error out"=w160:errorcluster)  [unwired: 12 in]
  n171 = call <vilib>:"DAQmx Clear Task.vi"("task in"=w163, "error in"=w160) -> ("error out"=w50:errorcluster)  [unwired: 13 in]
  n172 = call <vilib>:"DAQmx Stop Task.vi"("task/channels in"=w47, "error in"=w50) -> ("task out"=w46:refnum<k21>, "error out"=w49:errorcluster)  [unwired: 12 in]
  n173 = call <vilib>:"DAQmx Clear Task.vi"("task in"=w46, "error in"=w49) -> ("error out"=w48:errorcluster)  [unwired: 13 in]
  n174 = Close File(refnum=w140, error in=w48) -> (error out=w132:errorcluster)  [unwired: 1 out]
  n175 = Close File(refnum=w139, error in=w132) -> (error out=w131:errorcluster)  [unwired: 1 out]
  n176 = Close File(refnum=w138, error in=w131) -> (error out=w63:errorcluster)  [unwired: 1 out]
  n177 = Close File(refnum=w64, error in=w63) -> (error out=w62:errorcluster)  [unwired: 1 out]
  n178 = call-poly <vilib>:"DAQmx Write.vi"("task/channels in"=w100, "data"=0.0, "error in"=w62) -> ("task out"=w99:refnum<k21>, "error out"=w97:errorcluster)  [unwired: 10 in, 1 out]
  n179 = call <vilib>:"DAQmx Stop Task.vi"("task/channels in"=w99, "error in"=w97) -> ("task out"=w98:refnum<k21>, "error out"=w96:errorcluster)  [unwired: 12 in]
  n180 = call <vilib>:"DAQmx Clear Task.vi"("task in"=w98, "error in"=w96) -> ("error out"=w30:errorcluster)  [unwired: 13 in]
  n181 = call <vilib>:"DAQmx Stop Task.vi"("task/channels in"=w80, "error in"=w30) -> ("task out"=w84:refnum<k21>, "error out"=w83:errorcluster)  [unwired: 12 in]
  n182 = call <vilib>:"DAQmx Clear Task.vi"("task in"=w84, "error in"=w83) -> ("error out"=w27:errorcluster)  [unwired: 13 in]
  n183 = call <vilib>:"DAQmx Stop Task.vi"("task/channels in"=w26, "error in"=w27) -> ("task out"=w29:refnum<k21>, "error out"=w28:errorcluster)  [unwired: 12 in]
  n184 = call <vilib>:"DAQmx Clear Task.vi"("task in"=w29, "error in"=w28) -> ("error out"=w4:errorcluster)  [unwired: 13 in]
  n185 = call <vilib>:"DAQmx Stop Task.vi"("task/channels in"=w2, "error in"=w4) -> ("task out"=w6:refnum<k21>, "error out"=w5:errorcluster)  [unwired: 12 in]
  n186 = call <vilib>:"DAQmx Clear Task.vi"("task in"=w6, "error in"=w5) -> ("error out"=w3:errorcluster)  [unwired: 13 in]
  n187 = call <vilib>:"Simple Error Handler.vi"("error in (no error)"=w3) -> ()  [unwired: 4 in, 5 out]
